vi "MODBUS FACTORRY IO.vi"() -> ()   [LabVIEW 2020]
uses:
  <vilib>/Modbus/master/Create Master Instance (TCP).vi
  <vilib>/Modbus/master/Modbus Master.lvclass
panel:
  out "Boolean 11":bool
  out "Boolean 10":bool
  out "Boolean 9":bool
  out "Boolean 8":bool
  out "Boolean 7":bool
  in  "Boolean 6":bool
  in  "Boolean 5":bool
  in  "Boolean 4":bool
  in  "Boolean 3":bool
  in  "Boolean 2":bool
  in  "Boolean":bool
  out "REALIMENTE":u16(knob) scale=0.0..100.0
  out "SALIDA1":u16(knob) scale=0.0..100.0
  in  "VAR 2":u16(slide) scale=0.0..100.0
  in  "VAR":u16(slide) scale=0.0..100.0
  in  "stop":bool
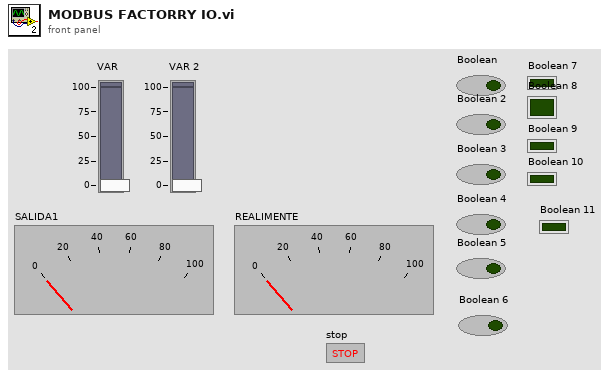
[diagram p1: front panel]
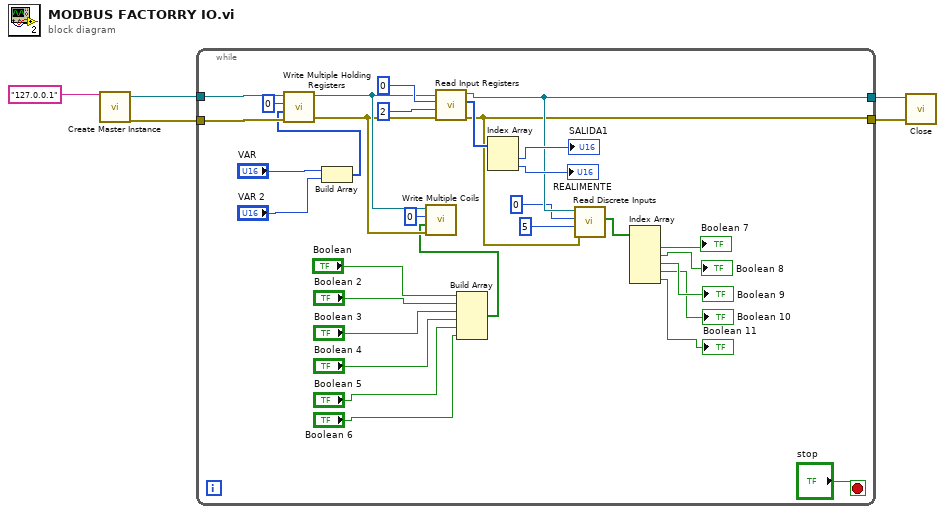
[diagram p0: block diagram]
diagram:
  n1 = call-poly <vilib>:"Create Master Instance.vi"("address"="127.0.0.1") -> ("error out"=w3:errorcluster, "TCP master instance"=w4:refnum<class "Modbus Master.lvclass">)  [unwired: 9 in]
  n2 = while {
    tunnel: w4 -> [w36]
    tunnel: w3 -> [w35]
    tunnel: [w15] -> w2
    tunnel: [w14] -> w1
    stop <- "stop" stop-if-true
    n3 = Build Array("VAR", "VAR 2") -> (w31:u16[])
    n4 = call-dynamic "Write Multiple Holding Registers.vi"("error in (no error)"=w35, "holding register values"=w31, "starting address"=u16 0, "Modbus master in"=w36) -> ("error out"=w24:errorcluster, "Modbus master out"=w25:refnum<class "Modbus Master.lvclass">)  [unwired: 6 in]
    n5 = call-dynamic "Read Input Registers.vi"("error in (no error)"=w24, "number of input registers"=u16 2, "starting address"=u16 0, "Modbus master in"=w25) -> ("error out"=w14:errorcluster, "register values"=w28:u16[], "Modbus master out"=w15:refnum<class "Modbus Master.lvclass">)  [unwired: 5 in]
    n6 = Build Array("Boolean", "Boolean 2", "Boolean 3", "Boolean 4", "Boolean 5", "Boolean 6") -> (w16:bool[])
    n7 = call-dynamic "Write Multiple Coils.vi"("error in (no error)"=w24, "coil values"=w16, "starting address"=u16 0, "Modbus master in"=w25) -> ()  [unwired: 6 in, 2 out]
    n8 = Index Array(array=w28) -> (element #1=→"SALIDA1":u16, element #2=→"REALIMENTE":u16)  [unwired: 2 in]
    n9 = call-dynamic "Read Discrete Inputs.vi"("error in (no error)"=w14, "number of discrete inputs"=u16 5, "starting address"=u16 0, "Modbus master in"=w15) -> ("discrete input values"=w11:bool[])  [unwired: 5 in, 2 out]
    n10 = Index Array(array=w11) -> (element #1=→"Boolean 7":bool, element #2=→"Boolean 8":bool, element #3=→"Boolean 9":bool, element #4=→"Boolean 10":bool, element #5=→"Boolean 11":bool)  [unwired: 5 in]
  }
  n11 = call-dynamic "Close.vi"("error in (no error)"=w1, "Modbus master in"=w2) -> ()  [unwired: 9 in, 1 out]
